vi "existance_filecheck.vi"(10 "selected EX":string[](array[string]), 11 "folder names":string[](array[string])) -> (0 "element":string, 3 "Array 3":cluster{string, bool}[](array[cluster]))   [LabVIEW 2018]
panel:
  out "Numeric":i32
  out "Array":bool[](array[boolean])
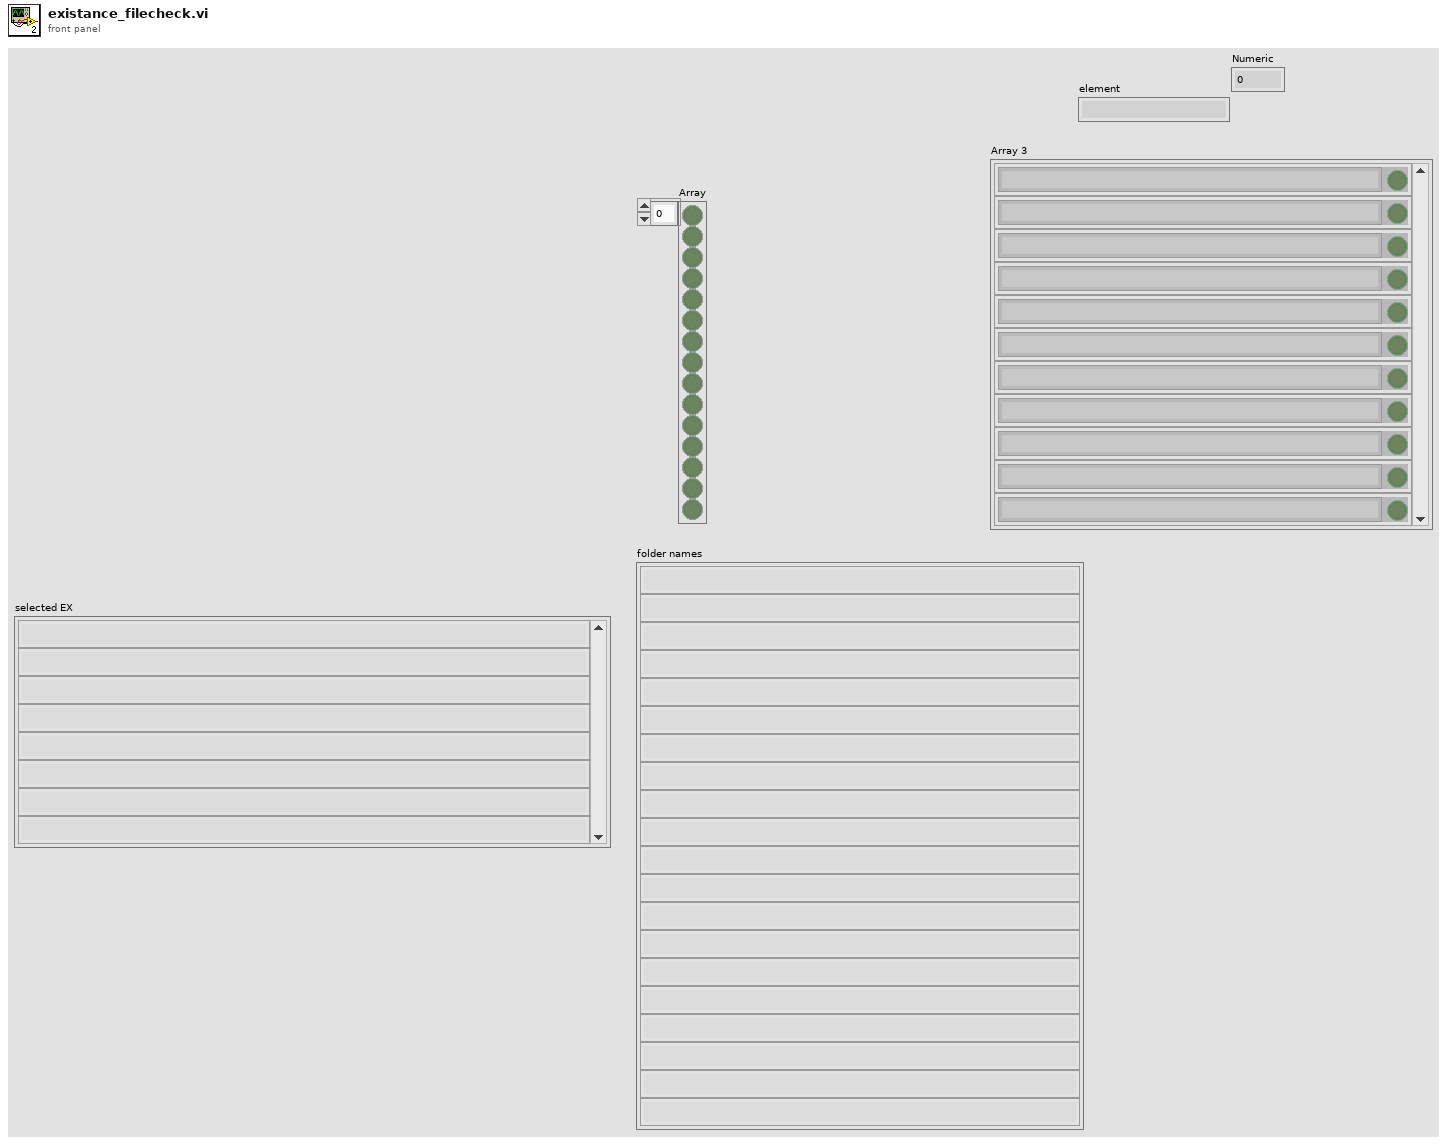
[diagram p1: front panel]
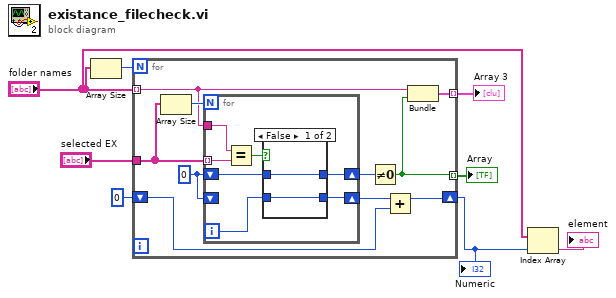
[diagram p0: block diagram]
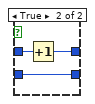
[diagram p2: hidden frame]
diagram:
  n1 = Array Size(array="folder names") -> (size(s)=w8:i32)
  n2 = for {
    N: w8 -> [_]
    tunnel: "selected EX" -> [w17]
    tunnel: "folder names" -> [w15] mode=indexing
    tunnel: [w14] -> w7 mode=indexing
    tunnel: [w13] -> w6 mode=indexing
    shift-right: [w10] -> w2
    shift-left: 0 -> [w9]
    w12 = 0
    n3 = Array Size(array=w17) -> (size(s)=w18:i32)
    n4 = for {
      N: w18 -> [_]
      tunnel: w15 -> [w25]
      tunnel: w17 -> [w24] mode=indexing
      shift-right: [w22] -> w16
      shift-left: w12 -> [w21]
      shift-right: [w19] -> w11
      shift-left: w12 -> [_]
      i -> [w20]
      n5 = Equal?(x=w25, y=w24) -> (x = y?=w23:bool)
      n6 = case shown="False" w23 {
        tunnel: [w27 w30] -> w22
        tunnel: w21 -> [w27 w29]
        tunnel: w20 -> [w26 w28]
        tunnel: [w26 w28] -> w19
        frame False {
        }
        frame True {
          n7 = Increment(x=w29) -> (x+1=w30:i32)
        }
      }
    }
    n8 = Not Equal To 0?(x=w16) -> (x != 0?=w13:bool)
    n9 = Add(x=w11, y=w9) -> (x+y=w10:i32)
    n10 = Bundle(w15, w13) -> (w14:cluster{string, bool})  [unwired: 1 in]
  }
  "Array 3" <- w7
  "Array" <- w6
  "Numeric" <- w2
  n11 = Index Array(array="folder names", index=w2) -> (element=→"element":string)
